vi "MotionProfileWriter.vi"(0 "PhoenixMotorControlDevRef":T6={"DeviceStatus"={"status"=FALSE, "code"=0, "source"=""}, "Type"=enum."PWM", "PWM"={"PWM Channel"=enum."Invalid", "DeadBand"={"Name"="", "maxPositivePwm"=0, "minPositivePwm"=0, "centerPwm"=0, "maxNegativePwm"=0, "minNegativePwm"=0, "angularRange"=0}}, "CAN"={"Device Number"=0, "SetOutput VI Ref"=variant(enum8{"Percent VBus", "Current", "Speed", "Position", "Voltage"} enum."Percent VBus"), "GetOutput VI Ref"=variant(refnum<k1> refnum), "Enable VI Ref"=variant(dbl 12.0), "Disable VI Ref"=variant(enum8{"Percent VBus", "Speed", "Position", "Slave", "Unchanged / Invalid", "Voltage Compensation", "Current", "Motion Profile"} enum."Percent VBus"), "Data"=variant}, "Invert"=FALSE, "DIO PWM"={"PWM \"Enable\" Channel"=enum."Invalid", "DIOChannel"=enum."Invalid", "PWM Rate"=0.0}}, 1 "ClearExistingMotionProfile":bool, 5 "Trajectory Points":T10[](array[typedef]) {"Time (ms)" items=["TrajectoryDuration_0ms"=0, "TrajectoryDuration_5ms"=5, "TrajectoryDuration_10ms"=10, "TrajectoryDuration_20ms"=20, "TrajectoryDuration_30ms"=30, "TrajectoryDuration_40ms"=40, "TrajectoryDuration_50ms"=50, "TrajectoryDuration_100ms"=100]}, 7 "MotorConfig":T1={"CAN Address"=0, "Invert"=FALSE, "InvertSensor"=FALSE, "Unit Conversion Factor"=0.0, "Brake Mode"=enum."Override to Brake", "Reverse Limt Switch Mode"=enum."Disabled", "Forward Limt Swith Mode"=enum."Disabled", "PWM Channel"=enum."Invalid", "Motor Controller Type"=enum."Talon SRX", "Peak Current (A)"=0, "Continuous Current (A)"=0, "Peak Duration (ms)"=0, "Current Limit Enable"=FALSE}, 9 "ProfileSlot0":i32, 11 "profileSlot1":i32, 12 "startIndex":i32) -> (4 "PhoenixMotorControlDevRef Out":T6={"DeviceStatus"={"status"=FALSE, "code"=0, "source"=""}, "Type"=enum."PWM", "PWM"={"PWM Channel"=enum."Invalid", "DeadBand"={"Name"="", "maxPositivePwm"=0, "minPositivePwm"=0, "centerPwm"=0, "maxNegativePwm"=0, "minNegativePwm"=0, "angularRange"=0}}, "CAN"={"Device Number"=0, "SetOutput VI Ref"=variant(enum8{"Percent VBus", "Current", "Speed", "Position", "Voltage"} enum."Percent VBus"), "GetOutput VI Ref"=variant(refnum<k1> refnum), "Enable VI Ref"=variant(dbl 12.0), "Disable VI Ref"=variant(enum8{"Percent VBus", "Speed", "Position", "Slave", "Unchanged / Invalid", "Voltage Compensation", "Current", "Motion Profile"} enum."Percent VBus"), "Data"=variant}, "Invert"=FALSE, "DIO PWM"={"PWM \"Enable\" Channel"=enum."Invalid", "DIOChannel"=enum."Invalid", "PWM Rate"=0.0}}, 15 "endIndex":i32)   [LabVIEW 2018, in "ArgosLib.lvlib"]
uses:
  ArgosLib.lvlib
  TypeDefs/TrajectoryPoint.ctl
  <vilib>/Rock Robotics/WPI/ThirdParty/Phoenix-LabVIEW/Motor Controller/Controls/CTRE_Phoenix_MotorControl_TrajectoryPointTimeDur.ctl
  <vilib>/Rock Robotics/WPI/MotorControl/WPI_MotorControlDeviceRef.ctl
  <vilib>/Rock Robotics/WPI/MotorControl/WPI_MotorControlType.ctl
  <vilib>/Rock Robotics/SystemInterfaces/DIO/FPGA_DIOPWMChannel.ctl
  <vilib>/Rock Robotics/WPI/PWM/WPI_PWMDeadband.ctl
  <vilib>/Rock Robotics/SystemInterfaces/DIO/FPGA_DIOChannel.ctl
  Config/ConfigComponents/TypeDefs/Config_Motor.ctl
  <vilib>/Rock Robotics/WPI/ThirdParty/Phoenix-LabVIEW/Motor Controller/Controls/CTRE_Phoenix_MotorControl_NeutralMode.ctl
  <vilib>/Rock Robotics/WPI/ThirdParty/Phoenix-LabVIEW/Motor Controller/Controls/CTRE_Phoenix_MotorControl_LimitSwitchNormal.ctl
  Config/ConfigComponents/TypeDefs/Config_MotorCtrlType.ctl
  <vilib>/Playing With Fusion Inc/Playing With Fusion Lib for FRC/PWF_Venom_LabVIEW/Public/TypeDefs/PwF_Venom_MPPoint.ctl
  <vilib>/Playing With Fusion Inc/Playing With Fusion Lib for FRC/PWF_Venom_LabVIEW/PwF_Venom.lvlib
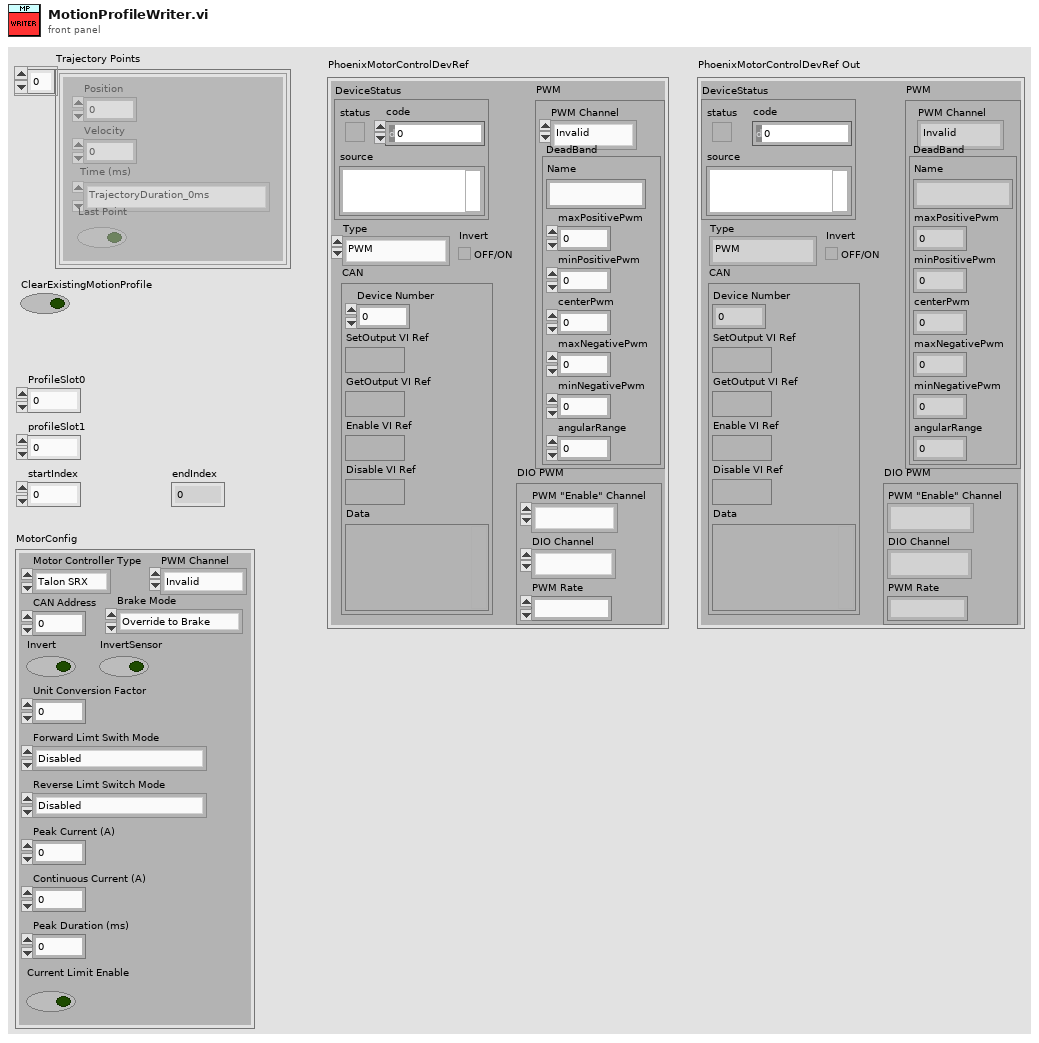
[diagram p1: front panel]
types:
  T1 = typedef "ArgosLib.lvlib/Config_Motor.ctl" = cluster{"CAN Address":u8, "Invert":bool, "InvertSensor":bool, "Unit Conversion Factor":dbl, "Brake Mode":T2, "Reverse Limt Switch Mode":T3, "Forward Limt Swith Mode":T3, "PWM Channel":T4, "Motor Controller Type":T5, "Peak Current (A)":i32, "Continuous Current (A)":i32, "Peak Duration (ms)":i32, "Current Limit Enable":bool}
  T2 = typedef "CTRE_Phoenix_MotorControl_NeutralMode.ctl" = enum8{"EEPROMSetting", "Override to Coast", "Override to Brake"}
  T3 = typedef "CTRE_Phoenix_MotorControl_LimitSwitchNormal.ctl" = enum16{"Normally Open", "Normally Closed", "Disabled"}
  T4 = typedef "FPGA_DIOPWMChannel.ctl" = enum8{"PWM 0", "PWM 1", "PWM 2", "PWM 3", "PWM 4", "PWM 5", "PWM 6", "PWM 7", "PWM 8", "PWM 9", "PWM MXP 0", "PWM MXP 1", "PWM MXP 2", "PWM MXP 3", "PWM MXP 4", "PWM MXP 5", "PWM MXP 6", "PWM MXP 7", "PWM MXP 8", "PWM MXP 9", "Invalid"}
  T5 = typedef "ArgosLib.lvlib/Config_MotorCtrlType.ctl" = enum16{"Disabled", "Talon SRX", "Talon SR", "Venom"}
  T6 = typedef "WPI_MotorControlDeviceRef.ctl" = cluster{"DeviceStatus":errorcluster, "Type":T7, "PWM":cluster{"PWM Channel":T4, "DeadBand":T8}, "CAN":cluster{"Device Number":u8, "SetOutput VI Ref":variant, "GetOutput VI Ref":variant, "Enable VI Ref":variant, "Disable VI Ref":variant, "Data":variant}, "Invert":bool, "DIO PWM":cluster{"PWM \"Enable\" Channel":T4, "DIOChannel":T9, "PWM Rate":dbl}}
  T7 = typedef "WPI_MotorControlType.ctl" = enum16{"PWM", "CAN", "DIO PWM"}
  T8 = typedef "WPI_PWMDeadband.ctl" = cluster{"Name":string, "maxPositivePwm":i32, "minPositivePwm":i32, "centerPwm":i32, "maxNegativePwm":i32, "minNegativePwm":i32, "angularRange":u16}
  T9 = typedef "FPGA_DIOChannel.ctl" = enum8{"DIO 0", "DIO 1", "DIO 2", "DIO 3", "DIO 4", "DIO 5", "DIO 6", "DIO 7", "DIO 8", "DIO 9", "DIO MXP 0", "DIO MXP 1", "DIO MXP 2", "DIO MXP 3", "DIO MXP 4", "DIO MXP 5", "DIO MXP 6", "DIO MXP 7", "DIO MXP 8", "DIO MXP 9", "DIO MXP 10", "DIO MXP 11", "DIO MXP 12", "DIO MXP 13", "DIO MXP 14", "DIO MXP 15", "SPI Port CS1", "SPI Port CS2", "SPI Port CS3", "SPI Port MISO", "SPI Port MOSI", "Invalid"}
  T10 = typedef "ArgosLib.lvlib/TrajectoryPoint.ctl" = cluster{"Position ":dbl, "Velocity ":dbl, "Time (ms)":T11, "Last Point":bool}
  T11 = typedef "CTRE_Phoenix_MotorControl_TrajectoryPointTimeDur.ctl" = i32
  T12 = cluster{"Top Buffer Remaining":i32, "Top Buffer Count":i32, "Bottom Buffer Count":i32, "Has Underrun?":bool, "Is Underrun?":bool, "Active Point Valid?":bool, "Is Last?":bool, "Profile Slot Select 0":i32, "Output Enable":i32, "Time Duration (ms)":i32, "Profile Slot Select 1":i32}
  T13 = typedef "PlayingWithFusionLib.lvlib/PwF_Venom.lvlib/PwF_Venom_MPPoint.ctl" = cluster{"Time":dbl, "Speed":dbl, "Position":dbl}
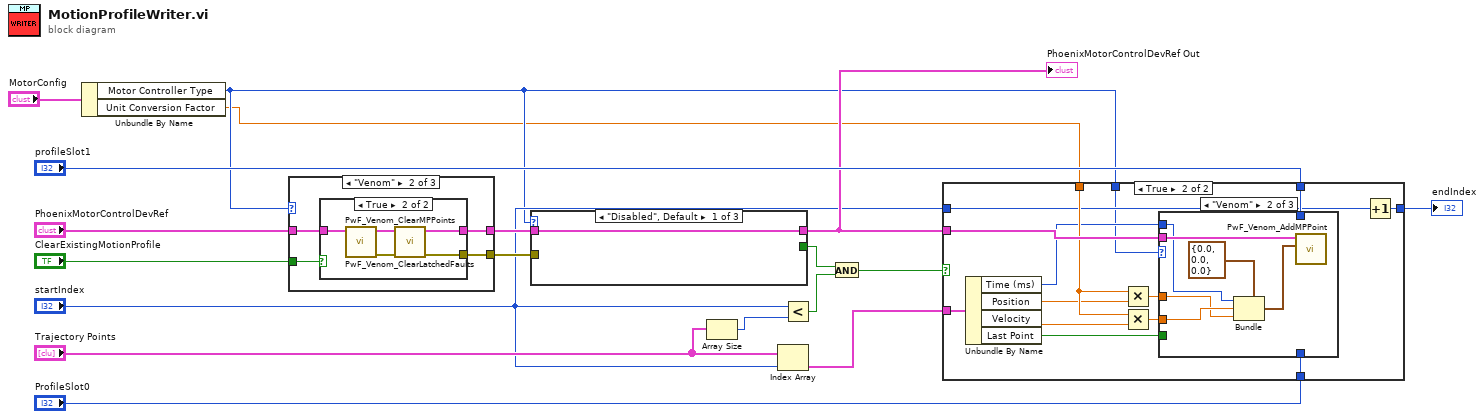
[diagram p0: block diagram]
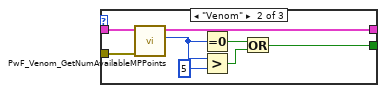
[diagram p2: hidden frame]
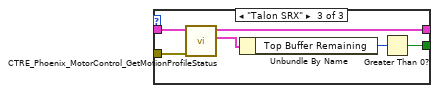
[diagram p3: hidden frame]
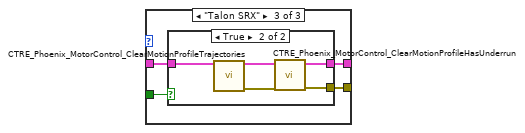
[diagram p6: hidden frame]
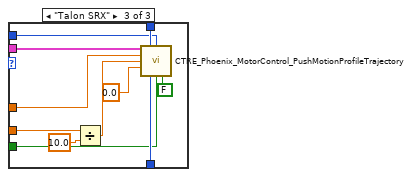
[diagram p10: hidden frame]
diagram:
  n1 = Unbundle By Name("MotorConfig") -> ("Motor Controller Type"=w2:T5, "Unit Conversion Factor"=w1:dbl)
  n2 = case shown="\"Venom\"" w2 {
    tunnel: "ClearExistingMotionProfile" -> [_ w20 w33]
    tunnel: "PhoenixMotorControlDevRef" -> [w19 w23 w32]
    tunnel: [w19 w22 w31] -> w14
    tunnel: [_ w21 w30] -> w13
    frame "Disabled", Default {
    }
    frame "Venom" {
      n3 = case shown="True" w20 {
        tunnel: w23 -> [w24 w29]
        tunnel: [w24 w25] -> w22
        tunnel: [_ w26] -> w21
        frame False {
        }
        frame True {
          n4 = call <vilib>:"PwF_Venom_ClearMPPoints.vi"("PwFVenomDevRefIn"=w29) -> ("error out"=w28:errorcluster, "PwFVenomDevRefOut"=w27:T6)  [unwired: 9 in]
          n5 = call <vilib>:"PwF_Venom_ClearLatchedFaults.vi"("error in"=w28, "PwFVenomDevRefIn"=w27) -> ("error out"=w26:errorcluster, "PwFVenomDevRefOut"=w25:T6)  [unwired: 8 in]
        }
      }
    }
    frame "Talon SRX" {
      n6 = case shown="True" w33 {
        tunnel: w32 -> [w34 w39]
        tunnel: [w34 w35] -> w31
        tunnel: [_ w36] -> w30
        frame False {
        }
        frame True {
          n7 = call <vilib>:"CTRE_Phoenix_MotorControl_ClearMotionProfileTrajectories.vi"("PhoenixMotorControlDevRef"=w39) -> ("PhoenixMotorControlDevRef"=w38:T6, "error out"=w37:errorcluster)  [unwired: 13 in]
          n8 = call <vilib>:"CTRE_Phoenix_MotorControl_ClearMotionProfileHasUnderrun.vi"("error in"=w37, "PhoenixMotorControlDevRef"=w38) -> ("error out"=w36:errorcluster, "PhoenixMotorControlDevRef"=w35:T6)  [unwired: 8 in]
        }
      }
    }
  }
  n9 = case shown="\"Disabled\", Default" w2 {
    tunnel: w14 -> [w40 w47 w54]
    tunnel: w13 -> [_ w48 w52]
    tunnel: [w40 w46 w51] -> w12
    tunnel: [_ w41 w49] -> w5
    frame "Disabled", Default {
    }
    frame "Venom" {
      n10 = call <vilib>:"PwF_Venom_GetNumAvailableMPPoints.vi"("error in"=w48, "PwFVenomDevRefIn"=w47) -> ("Available MP Points"=w43:u16, "PwFVenomDevRefOut"=w46:T6)  [unwired: 7 in, 1 out]
      n11 = Equal To 0?(x=w43) -> (x = 0?=w45:bool)
      n12 = Greater?(x=w43, y=u16 5) -> (0:w44:bool)
      n13 = Or(x=w45, y=w44) -> (x .or. y?=w41:bool)
    }
    frame "Talon SRX" {
      n14 = call <vilib>:"CTRE_Phoenix_MotorControl_GetMotionProfileStatus.vi"("error in"=w52, "PhoenixMotorControlDevRef"=w54) -> ("Motion Profile Status"=w53:T12, "PhoenixMotorControlDevRef"=w51:T6)  [unwired: 7 in, 1 out]
      n15 = Unbundle By Name(w53) -> ("Top Buffer Remaining"=w50:i32)
      n16 = Greater Than 0?(x=w50) -> (x > 0?=w49:bool)
    }
  }
  "PhoenixMotorControlDevRef Out" <- w12
  n17 = Array Size(array="Trajectory Points") -> (size(s)=w8:i32)
  n18 = Index Array(array="Trajectory Points", index="startIndex") -> (element=w11:T10)
  n19 = Less?(x="startIndex", y=w8) -> (x < y?=w6:bool)
  n20 = And(x=w5, y=w6) -> (x .and. y?=w4:bool)
  n21 = case shown="True" w4 {
    tunnel: "ProfileSlot0" -> [_ w69]
    tunnel: "profileSlot1" -> [_ w68]
    tunnel: w12 -> [_ w67]
    tunnel: w1 -> [_ w66]
    tunnel: w11 -> [_ w59]
    tunnel: "startIndex" -> [w55 w58]
    tunnel: [w55 w57] -> w10
    tunnel: w2 -> [_ w56]
    frame False {
    }
    frame True {
      n22 = Unbundle By Name(w59) -> ("Time (ms)"=w64:T11, "Position"=w62:dbl, "Velocity"=w61:dbl, "Last Point"=w65:bool)
      n23 = Multiply(x=w66, y=w62) -> (x*y=w63:dbl)
      n24 = Multiply(x=w66, y=w61) -> (x*y=w60:dbl)
      n25 = case shown="\"Venom\"" w56 {
        tunnel: w69 -> [_ _ w86]
        tunnel: w68 -> [_ _ w85]
        tunnel: w67 -> [_ w75 w84]
        tunnel: w65 -> [_ _ w83]
        tunnel: w64 -> [_ w71 w82]
        tunnel: w63 -> [_ w72 w79]
        tunnel: w60 -> [_ w73 w77]
        frame "Disabled", Default {
        }
        frame "Venom" {
          n26 = Bundle(cluster=T13 {"Time"=0.0, "Speed"=0.0, "Position"=0.0} ("Motion Profile Point"), "Time"=w71, "Speed"=w73, "Position"=w72) -> (w70:T13)
          n27 = call <vilib>:"PwF_Venom_AddMPPoint.vi"("Motion Profile Point"=w70, "PwFVenomDevRefIn"=w75) -> ()  [unwired: 8 in, 2 out]
        }
        frame "Talon SRX" {
          n28 = Divide(x=w77, y=10.0) -> (x/y=w76:dbl)
          n29 = call <vilib>:"CTRE_Phoenix_MotorControl_PushMotionProfileTrajectory.vi"("PhoenixMotorControlDevRef"=w84, "profileSlotSelect1"=w85, "durationMs"=w82, "position"=w79, "velocity"=w76, "auxiliaryPos"=0.0 ("headingDeg"), "profileSlotSelect0"=w86, "isLastPoint?"=w83, "Zero Position?"=FALSE) -> ()  [unwired: 5 in, 2 out]
        }
      }
      n30 = Increment(x=w58) -> (x+1=w57:i32)
    }
  }
  "endIndex" <- w10
